vi "Launch Async Job.vi"(6 "timeout (500 ms)":i32=500, 8 "error in (no error)":errorcluster, 10 "stdin":string, 11 "Job in":refnum<class "Job.lvclass">) -> (0 "error out":errorcluster, 1 "exception":i32, 2 "Job GUID":string, 3 "Job out":refnum<class "Job.lvclass">)   [LabVIEW 2013, in "openCronJob.lvlib" / "Job.lvclass"]
uses:
  Job.lvclass
  Job Details -- cluster.ctl
  Job.lvclass/Job.ctl
  JobReport/JobReport.lvclass
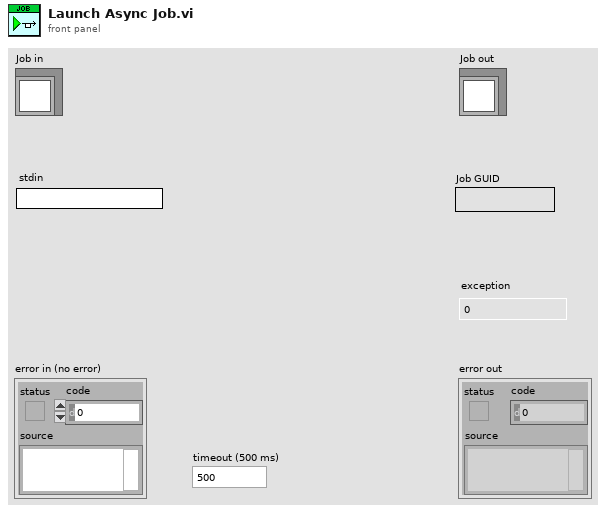
[diagram p1: front panel]
types:
  T1 = typedef "openCronJob.lvlib/Job.lvclass/Job Details -- cluster.ctl" = cluster{"Name":string, "GUID":string, "Abort":refnum<notifier>}
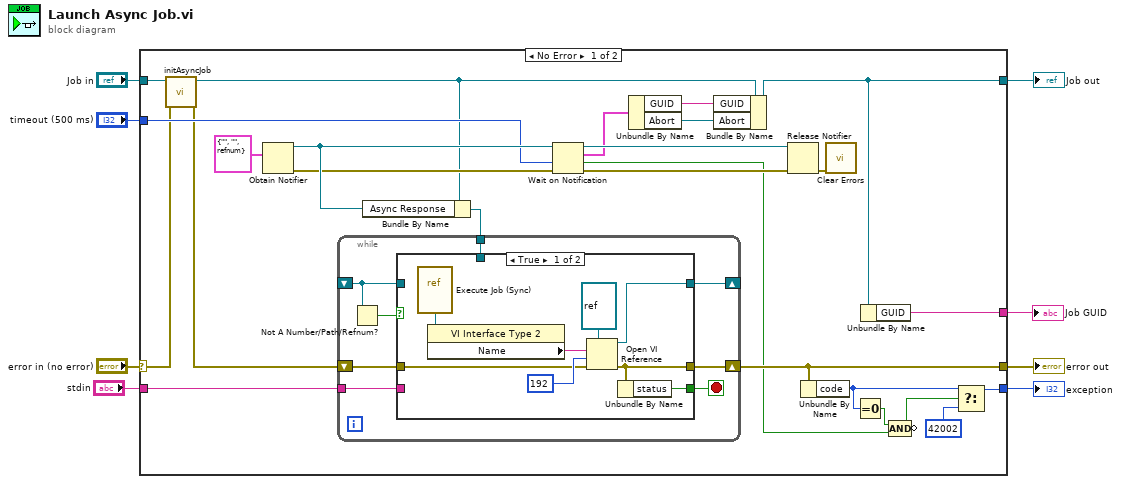
[diagram p0: block diagram]
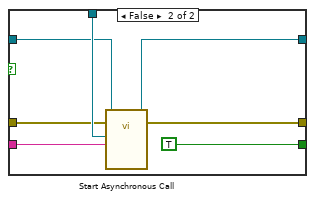
[diagram p2: hidden frame]
diagram:
  n1 = case shown="No Error" "error in (no error)" {
    selector: "error in (no error)" -> [w12 w58]
    tunnel: [w28 w58] -> w5
    tunnel: [w16 w57] -> w6
    tunnel: "Job in" -> [w13 w57]
    tunnel: [w26 _] -> w4
    tunnel: "timeout (500 ms)" -> [w21 _]
    tunnel: [w15 _] -> w2
    tunnel: "stdin" -> [w10 _]
    frame No Error {
      n2 = call "initAsyncJob.vi"("error in (no error)"=w12, "Job in"=w13) -> ("error out"=w11:errorcluster, "Job out"=w14:refnum<class "Job.lvclass">)  [unwired: 8 in]
      n3 = Obtain Notifier(notification data type=T1 {"Name"="", "GUID"="", "Abort"=refnum} ("Job Details")) -> (notifier out=w33:refnum<notifier>, error out=w32:errorcluster)  [unwired: 3 in, 1 out]
      n4 = Bundle By Name(cluster=w14, "Async Response"=w33) -> (w9:refnum<class "Job.lvclass">)
      n5 = while {
        tunnel: w10 -> [w40]
        tunnel: w9 -> [w39]
        shift-right: [w38] -> _
        shift-left: _ -> [w34]
        shift-right: [w37] -> w28
        shift-left: w11 -> [w41]
        stop <- w36 stop-if-true
        n6 = Not A Number/Path/Refnum?(number/path/refnum=w34) -> (NaN/Path/Refnum?=w35:bool)
        n7 = case shown="True" w35 {
          tunnel: w41 -> [w46 w51]
          tunnel: w40 -> [_ w56]
          tunnel: w39 -> [_ w55]
          tunnel: [w42 w54] -> w38
          tunnel: [w43 w53] -> w37
          tunnel: [w44 TRUE ("status")] -> w36
          tunnel: w34 -> [_ w52]
          frame True {
            n8 = vi-ref "Execute Job (Sync).vi"() -> (w49:refnum<vi>)
            n9 = property class="VI Interface Type 2"(reference=w49) -> ("Name"=w48:string)  [unwired: 1 in, 2 out]
            n10 = Open VI Reference(type specifier VI Refnum (for type only)=refnum<vi> refnum, vi path=w48, options=192, error in (no error)=w46) -> (vi reference=w42:refnum<vi>, error out=w43:errorcluster)  [unwired: 2 in]
            n11 = Unbundle By Name(w43) -> ("status"=w44:bool)
          }
          frame False {
            n12 = call-by-ref "Start Asynchronous Call"(reference=w52, error in=w51, "stdin"=w56, "Job in"=w55) -> (reference out=w54:refnum<vi>, error out=w53:errorcluster)  [unwired: 6 in, 4 out]
          }
        }
      }
      n13 = Wait on Notification(notifier=w33, timeout in ms (-1)=w21, error in (no error)=w32) -> (notifier out=w31:refnum<notifier>, notification=w19:T1, timed out?=w24:bool, error out=w30:errorcluster)  [unwired: 1 in]
      n14 = Unbundle By Name(w19) -> ("GUID"=w18:string, "Abort"=w17:refnum<notifier>)
      n15 = Bundle By Name(cluster=w14, "GUID"=w18, "Abort"=w17) -> (w16:refnum<class "Job.lvclass">)
      n16 = Release Notifier(notifier=w31, error in (no error)=w30) -> (error out=w29:errorcluster)  [unwired: 1 in, 2 out]
      n17 = Unbundle By Name(w28) -> ("code"=w27:i32)
      n18 = call <vilib>:"Clear Errors.vi"("error in (no error)"=w29) -> ()  [unwired: 6 in, 1 out]
      n19 = Equal To 0?(x=w27) -> (x = 0?=w25:bool)
      n20 = Unbundle By Name(w16) -> ("GUID"=w15:string)
      n21 = Compound Arithmetic op=AND(w25, w24) -> (invert w23:bool)
      n22 = Select(t=w27, s=w23, f=42002 ("timeout in ms (-1)")) -> (s? t:f=w26:i32)
    }
    frame Error {
    }
  }
  "error out" <- w5
  "Job out" <- w6
  "exception" <- w4
  "Job GUID" <- w2
